vi "Plugin_Worker_Template.vi"(8 "error in (no error)":errorcluster={"status"=FALSE, "code"=0, "source"="\"\""}, 10 "cancel signal":string, 11 "PluginRequest":string) -> (0 "error out":errorcluster={"status"=FALSE, "code"=0, "source"="\"\""}, 2 "status ok":bool, 3 "Progress/status/result":string)   [LabVIEW 2026]
doc: "INTENT: Standard specialized operation implementation pattern. LOGIC: State-driven nonblocking work, request Bridge permissions, publish heartbeat and result, release on completion."
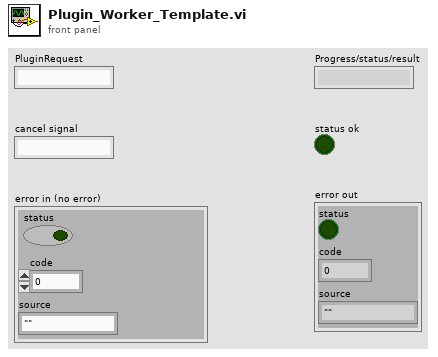
[diagram p1: front panel]
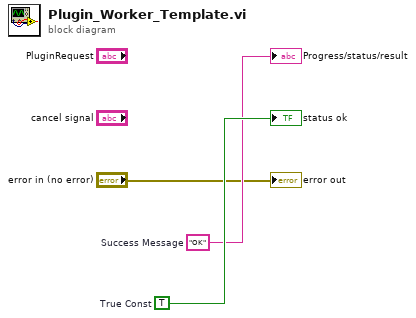
[diagram p0: block diagram]
diagram:
  w3 = TRUE  # True Const
  w2 = "OK"  # Success Message
  "Progress/status/result" <- w2
  "status ok" <- w3
  "error out" <- "error in (no error)"
